vi "libssh2_session_set_last_error.vi"(8 "error in (no error)":errorcluster, 9 "error message":string, 10 "error code":i32, 11 "session":T1) -> (0 "error out":errorcluster)   [LabVIEW 2017, in "libssh2.lvlib"]
doc: "Set the last error code and error message for a session."
uses:
  libssh2.lvlib
  Session Refnum.ctl
  Not A Session.vi
  <vilib>/Utility/error.llb/Error Cluster From Error Code.vi
  Global Settings.vi
  Read Session Refnum.vi
  <vilib>/Utility/semaphor.llb/Acquire Semaphore.vi
  <vilib>/Utility/semaphor.llb/Release Semaphore.vi
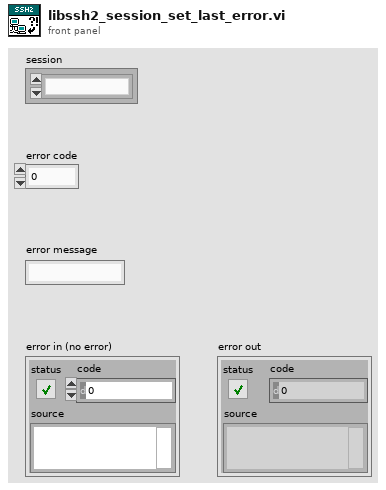
[diagram p1: front panel]
types:
  T1 = typedef "libssh2.lvlib/Session Refnum.ctl" = refnum<k1>
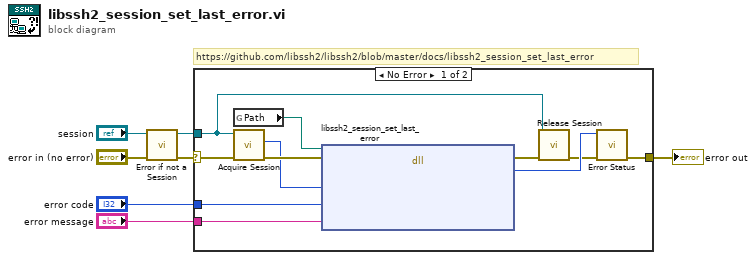
[diagram p0: block diagram]
diagram:
  # "https://github.com/libssh2/libssh2/blob/master/docs/libssh2_session_set_last_error"
  n1 = call "Error if not a Session.vi"("error in (no error)"="error in (no error)", "session"="session") -> ("error out"=w5:errorcluster, "session out"=w3:T1)  [unwired: 8 in]
  n2 = case shown="No Error" w5 {
    selector: w5 -> [w17 w19]
    tunnel: [w11 w19] -> w7
    tunnel: w3 -> [w8 _]
    tunnel: "error code" -> [w13 _]
    tunnel: "error message" -> [w12 _]
    frame No Error {
      n3 = global read "Global Settings.vi" "Path"() -> (w14:path)
      n4 = call "Acquire Session.vi"("error in (no error)"=w17, "session"=w8) -> ("error out"=w16:errorcluster, "LIBSSH2_SESSION*"=w15:u64)  [unwired: 7 in, 1 out]
      n5 = dll-call lib="?" fn="libssh2_session_set_last_error"(path in=w14, error in=w16, "session"=w15, "errcode"=w13, "errmsg"=w12) -> (error out=w18:errorcluster, "return value"=w10:i32)  [unwired: 4 in, 1 out]
      n6 = call "Release Session.vi"("error in (no error)"=w18, "session"=w8) -> ("error out"=w9:errorcluster)  [unwired: 9 in]
      n7 = call "Error Status.vi"("error in (no error)"=w9, "return value"=w10) -> ("error out"=w11:errorcluster)  [unwired: 8 in, 1 out]
    }
    frame Error {
    }
  }
  "error out" <- w7
